vi "reformat message.vi"(8 "error in (no error)":errorcluster, 11 "TCS in":refnum<class "TCS.lvclass">) -> (0 "error out":errorcluster, 3 "TCS out":refnum<class "TCS.lvclass">)   [LabVIEW 2018, in "TCS.lvclass"]
uses:
  TCS.lvclass
  <vilib>/Utility/error.llb/whitespace.ctl
  TCS.lvclass/TCS.ctl
  RxTx/RxTx.lvclass
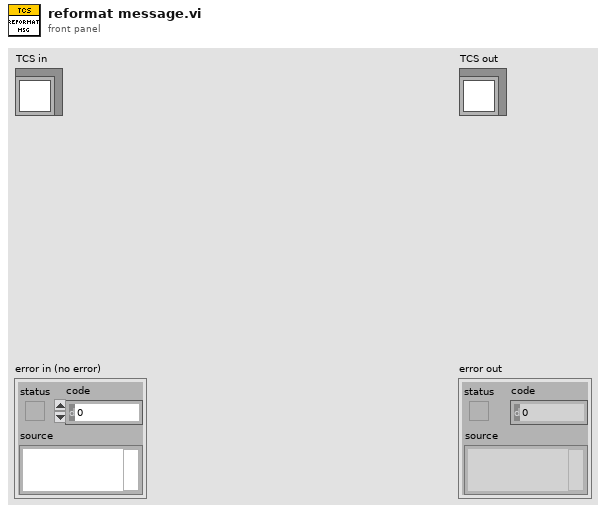
[diagram p1: front panel]
types:
  T1 = typedef "whitespace.ctl" = u16
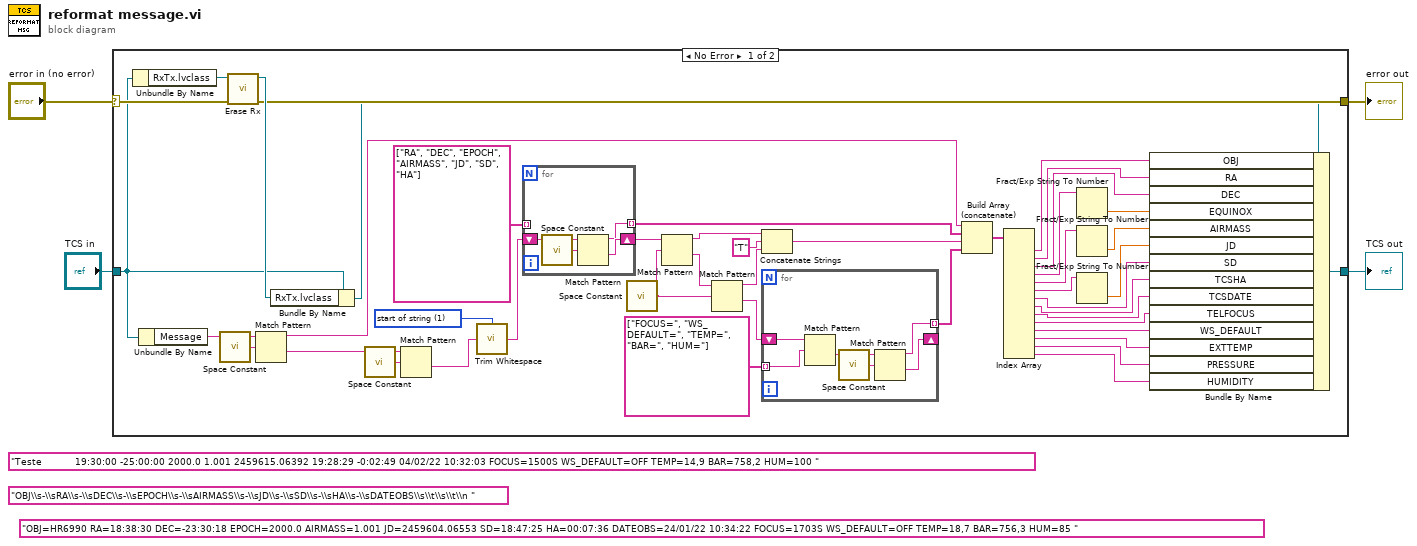
[diagram p0: block diagram]
diagram:
  (unwired) "Teste           19:30:00 -25:00:00 2000.0 1.001 2459615.06392 19:28:29 -0:02:49 04/02/22 10:32:03 FOCUS=1500S WS_DEFAULT=OFF TEMP=14,9 BAR=758,2 HUM=100 "
  (unwired) "OBJ=HR6990 RA=18:38:30 DEC=-23:30:18 EPOCH=2000.0 AIRMASS=1.001 JD=2459604.06553 SD=18:47:25 HA=00:07:36 DATEOBS=24/01/22 10:34:22 FOCUS=1703S WS_DEFAULT=OFF TEMP=18,7 BAR=756,3 HUM=85 "
  (unwired) "OBJ\\s-\\sRA\\s-\\sDEC\\s-\\sEPOCH\\s-\\sAIRMASS\\s-\\sJD\\s-\\sSD\\s-\\sHA\\s-\\sDATEOBS\\s\\t\\s\\t\\n "
  n1 = case shown="No Error" "error in (no error)" {
    selector: "error in (no error)" -> [w40 w61]
    tunnel: [w39 w61] -> w3
    tunnel: [w24 w60] -> w1
    tunnel: "TCS in" -> [w38 w60]
    frame No Error {
      w45 = T1 1 items=["both", "start of string", "end of string"] ("location (both)")
      n2 = Unbundle By Name(w38) -> ("RxTx.lvclass"=w42:refnum<class "RxTx.lvclass">)
      n3 = Unbundle By Name(w38) -> ("Message"=w5:string)
      n4 = call <vilib>:"Space Constant.vi"() -> ("String"=w48:string)
      n5 = call "Erase Rx.vi"("error in (no error)"=w40, "RxTx in"=w42) -> ("error out"=w39:errorcluster, "RxTx out"=w41:refnum<class "RxTx.lvclass">)  [unwired: 8 in]
      n6 = Match Pattern(string=w5, regular expression=w48) -> (before substring=w26:string, after substring=w47:string)  [unwired: 1 in, 2 out]
      n7 = Bundle By Name(cluster=w38, "RxTx.lvclass"=w41) -> (w25:refnum<class "TCS.lvclass">)
      n8 = call <vilib>:"Space Constant.vi"() -> ("String"=w46:string)
      n9 = Match Pattern(string=w47, regular expression=w46) -> (after substring=w44:string)  [unwired: 1 in, 3 out]
      n10 = call <vilib>:"Trim Whitespace.vi"("string"=w44, "location (both)"=w45) -> ("trimmed string"=w43:string)
      n11 = for {
        tunnel: string[] ["RA", "DEC", "EPOCH", "AIRMASS", "JD", "SD", "HA"] -> [_] mode=indexing
        shift-right: [w57] -> w37
        shift-left: w43 -> [w59]
        tunnel: [w56] -> w30 mode=indexing
        n12 = call <vilib>:"Space Constant.vi"() -> ("String"=w58:string)
        n13 = Match Pattern(string=w59, regular expression=w58) -> (before substring=w56:string, after substring=w57:string)  [unwired: 1 in, 2 out]
      }
      n14 = call <vilib>:"Space Constant.vi"() -> ("String"=w35:string)
      n15 = Match Pattern(string=w37, regular expression=w35) -> (before substring=w34:string, after substring=w36:string)  [unwired: 1 in, 2 out]
      n16 = Match Pattern(string=w36, regular expression=w35) -> (before substring=w32:string, after substring=w29:string)  [unwired: 1 in, 2 out]
      n17 = Concatenate Strings(w34, "T" ("string"), w32) -> (w31:string)
      n18 = for {
        tunnel: string[] ["FOCUS=", "WS_DEFAULT=", "TEMP=", "BAR=", "HUM="] -> [w54] mode=indexing
        shift-right: [w50] -> _
        shift-left: w29 -> [w55]
        tunnel: [w52] -> w27 mode=indexing
        n19 = Match Pattern(string=w55, regular expression=w54) -> (after substring=w51:string)  [unwired: 1 in, 3 out]
        n20 = call <vilib>:"Space Constant.vi"() -> ("String"=w53:string)
        n21 = Match Pattern(string=w51, regular expression=w53) -> (before substring=w52:string, after substring=w50:string)  [unwired: 1 in, 2 out]
      }
      n22 = Build Array (concatenate)(w26, w30, w31, w27) -> (w23:string[])
      n23 = Index Array(array=w23) -> (element #1=w22:string, element #2=w21:string, element #3=w20:string, element #4=w18:string, element #5=w16:string, element #6=w14:string, element #7=w13:string, element #8=w12:string, element #9=w11:string, element #10=w10:string, element #11=w9:string, element #12=w8:string, element #13=w7:string, element #14=w6:string)  [unwired: 14 in]
      n24 = Fract/Exp String To Number(string=w18) -> (number=w19:dbl)  [unwired: 3 in, 1 out]
      n25 = Fract/Exp String To Number(string=w16) -> (number=w17:dbl)  [unwired: 3 in, 1 out]
      n26 = Fract/Exp String To Number(string=w14) -> (number=w15:dbl)  [unwired: 3 in, 1 out]
      n27 = Bundle By Name(cluster=w25, "OBJ"=w22, "RA"=w21, "DEC"=w20, "EQUINOX"=w19, "AIRMASS"=w17, "JD"=w15, "SD"=w13, "TCSHA"=w12, "TCSDATE"=w11, "TELFOCUS"=w10, "WS_DEFAULT"=w9, "EXTTEMP"=w8, "PRESSURE"=w7, "HUMIDITY"=w6) -> (w24:refnum<class "TCS.lvclass">)
    }
    frame Error {
    }
  }
  "error out" <- w3
  "TCS out" <- w1
